vi "Fix_size_Template.vi"() -> ()   [LabVIEW 2012]
panel:
  out "Array_Out":variant[](array[variant])
  in  "Size":i32
  in  "Array_In":variant[](array[variant])
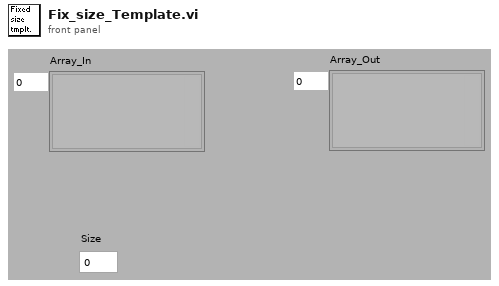
[diagram p1: front panel]
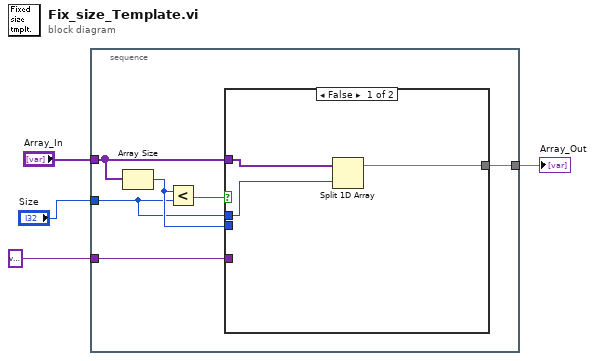
[diagram p0: block diagram]
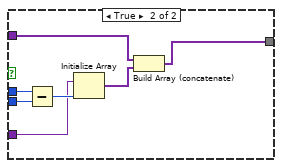
[diagram p2: hidden frame]
diagram:
  n1 = stacked-sequence {
    tunnel: "Array_In" -> [w6]
    tunnel: "Size" -> [w8]
    tunnel: variant ("Variant") -> [w7]
    tunnel: [w5] -> w1
    frame #0 {
      n2 = Array Size(array=w6) -> (size(s)=w9:i32)
      n3 = Less?(x=w9, y=w8) -> (x < y?=w10:bool)
      n4 = case shown="False" w10 {
        tunnel: w9 -> [_ w20]
        tunnel: w8 -> [w11 w19]
        tunnel: w7 -> [_ w17]
        tunnel: w6 -> [w13 w15]
        tunnel: [w12 w14] -> w5
        frame False {
          n5 = Split 1D Array(array=w13, index=w11) -> (first subarray=w12:variant[])  [unwired: 1 out]
        }
        frame True {
          n6 = Subtract(x=w19, y=w20) -> (x-y=w18:i32)
          n7 = Initialize Array(w17, w18) -> (w16:variant[])
          n8 = Build Array (concatenate)(w15, w16) -> (w14:variant[])
        }
      }
    }
  }
  "Array_Out" <- w1
